vi "Build_Row.vi"(8 "error in (no error)":errorcluster, 9 "Packet Number":i32, 11 "Ethernet frame":T1 {"fcs" format="%08x"; "network timestamp" format="%<%.7X\n%x>T"; "frame data" format="%x"; "local timestamp" format="%<%.7X\n%x>T"; "type" items=["Ethernet Data"=0, "Delay"=225, "Future Time Wait"=226]}) -> (0 "error out":errorcluster, 3 "Packet":string[](array[string]))   [LabVIEW 2025, in "Automotive Ethernet Bus Monitor.lvclass"]
uses:
  Automotive Ethernet Bus Monitor.lvclass
  <vilib>/xnet/xnet.llb/XNET Frame Ethernet.ctl
  <vilib>/xnet/xnet.llb/XNET Frame Type Ethernet.ctl
  Automotive Ethernet Bus Monitor UI/Automotive Ethernet Bus Monitor UI.lvlib
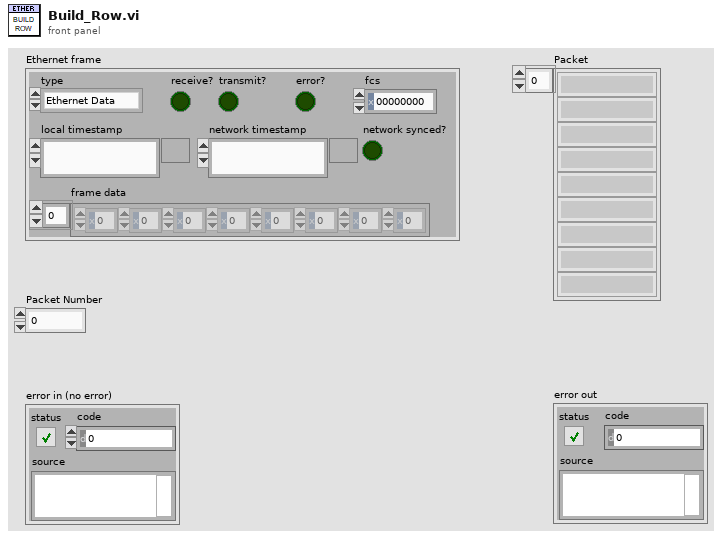
[diagram p1: front panel]
types:
  T1 = typedef "XNET Frame Ethernet.ctl" = cluster{"local timestamp":timestamp, "network timestamp":timestamp, "frame data":u8[], "fcs":u32, "type":T2, "network synced?":bool, "receive?":bool, "transmit?":bool, "error?":bool}
  T2 = typedef "XNET Frame Type Ethernet.ctl" = u16
  T3 = cluster{"destination MAC address":cluster{u8, u8, u8, u8, u8, u8}, "source MAC address":cluster{u8, u8, u8, u8, u8, u8}, "Has VLAN Tag":bool, "VLAN Tag":cluster{"TPID":u16, "priority":u8, "DEI":bool, "VID":u16}, "Ethertype":u16}
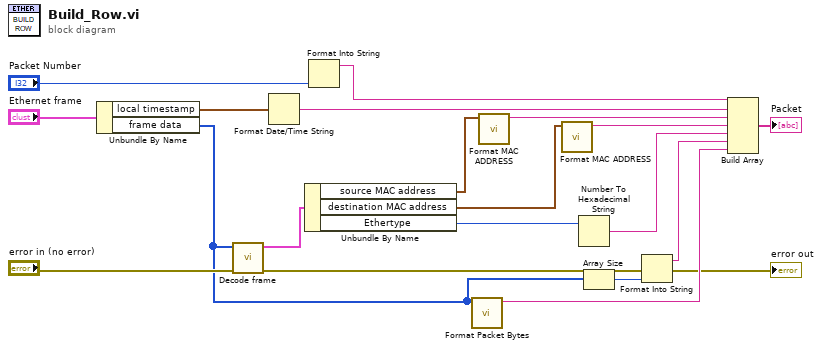
[diagram p0: block diagram]
diagram:
  n1 = Unbundle By Name("Ethernet frame") -> ("local timestamp"=w14:timestamp, "frame data"=w4:u8[])
  n2 = call "Decode frame.vi"("error in (no error)"="error in (no error)", "frame data"=w4) -> ("error out"=w3:errorcluster, "Ethernet Header Cluster"=w5:T3)  [unwired: 7 in, 1 out]
  n3 = Format Date/Time String(seconds (now)=w14) -> (date/time string=w19:string)  [unwired: 2 in]
  n4 = Unbundle By Name(w5) -> ("source MAC address"=w11:cluster{u8, u8, u8, u8, u8, u8}, "destination MAC address"=w9:cluster{u8, u8, u8, u8, u8, u8}, "Ethertype"=w1:u16)
  n5 = Format Into String("Packet Number") -> (resulting string=w20:string)  [unwired: 3 in, 1 out]
  n6 = call "Format Packet Bytes.vi"("frame data"=w4) -> ("spreadsheet string"=w7:string)  [unwired: 10 in]
  n7 = call "Format MAC ADDRESS.vi"("source MAC address"=w11) -> ("spreadsheet string"=w10:string)  [unwired: 10 in]
  n8 = call "Format MAC ADDRESS.vi"("source MAC address"=w9) -> ("spreadsheet string"=w8:string)  [unwired: 10 in]
  n9 = Number To Hexadecimal String(2:w1) -> (0:w16:string)  [unwired: 1 in]
  n10 = Array Size(array=w4) -> (size(s)=w18:i32)
  n11 = Format Into String(error in=w3, w18) -> (resulting string=w17:string, error out=→"error out":errorcluster)  [unwired: 2 in]
  n12 = Build Array(w20, w19, w10, w8, w16, w17, w7) -> (→"Packet":string[])
